vi "Init reg run.vi"() -> (1 "Rég acqui":T1(array[cluster]))   [LabVIEW 2022 SP3]
uses:
  Variables globales/Variables glob EUROTHERM.vi
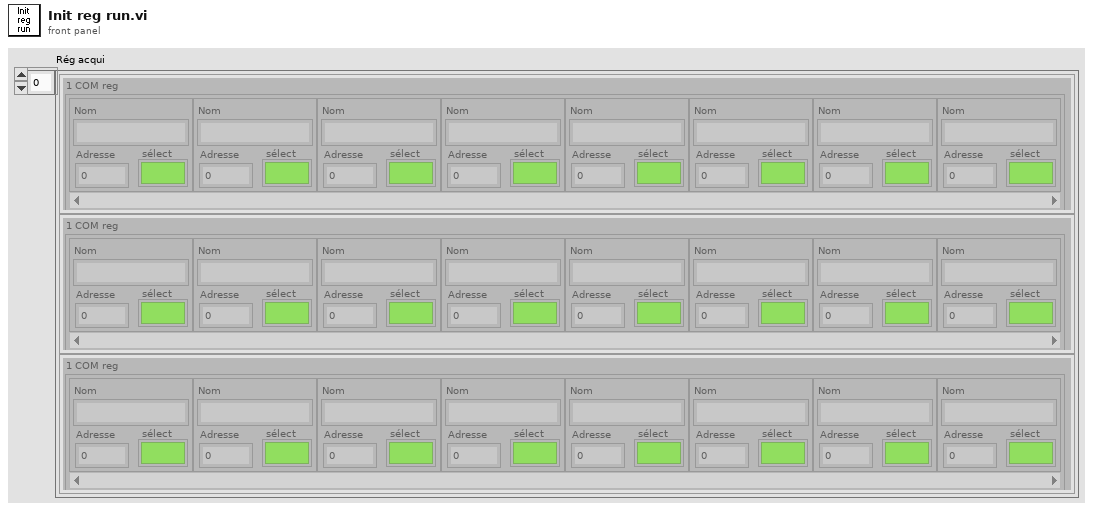
[diagram p1: front panel]
types:
  T1 = cluster{"1 COM reg":cluster{"Nom":string, "Adresse":u8, "sélect":bool}[]}[]
  T2 = cluster{"Noms voies select acqui 1COM":string[]}[]
  T3 = cluster{"1 COM reg":cluster{"Nom":string, "Adresse":u8, "sélect":bool}[]}
  T4 = cluster{"Nom":string, "Adresse":u8, "sélect":bool}[]
  T5 = cluster{"Nom":string, "Adresse":u8, "sélect":bool}
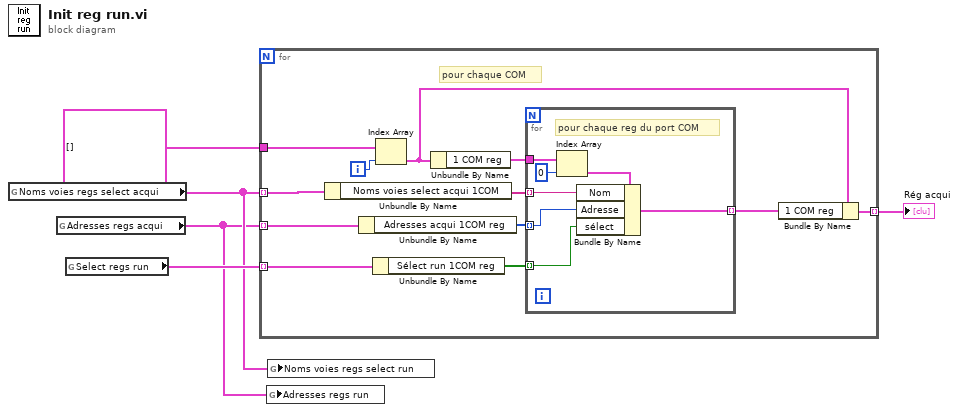
[diagram p0: block diagram]
diagram:
  n1 = global read "Variables glob EUROTHERM.vi" "Noms voies regs select acqui"() -> (w2:T2)
  n2 = global read "Variables glob EUROTHERM.vi" "Adresses regs acqui"() -> (w1:cluster{"Adresses acqui 1COM reg":u16[]}[])
  n3 = global read "Variables glob EUROTHERM.vi" "Select regs run"() -> (w3:cluster{"Sélect run 1COM reg":bool[]}[])
  n4 = for {
    tunnel: w2 -> [w11] mode=indexing
    tunnel: w1 -> [w13] mode=indexing
    tunnel: T1 [] ("Rég dispo") -> [w15]
    tunnel: [w16] -> w5 mode=indexing
    tunnel: w3 -> [w7] mode=indexing
    i -> [w14]
    # "pour chaque COM"
    n5 = Unbundle By Name(w11) -> ("Noms voies select acqui 1COM"=w10:string[])
    n6 = Unbundle By Name(w13) -> ("Adresses acqui 1COM reg"=w12:u16[])
    n7 = Unbundle By Name(w7) -> ("Sélect run 1COM reg"=w6:bool[])
    n8 = Index Array(array=w15, index=w14) -> (element=w8:T3)
    n9 = Unbundle By Name(w8) -> ("1 COM reg"=w17:T4)
    n10 = for {
      tunnel: w17 -> [w23]
      tunnel: w10 -> [w24] mode=indexing
      tunnel: w12 -> [w21] mode=indexing
      tunnel: [w20] -> w9 mode=indexing
      tunnel: w6 -> [w18] mode=indexing
      # "pour chaque reg du port COM"
      n11 = Index Array(array=w23, index=0 ("indice")) -> (element=w19:T5)
      n12 = Bundle By Name(cluster=w19, "Nom"=w24, "Adresse"=w21, "sélect"=w18) -> (w20:T5)
    }
    n13 = Bundle By Name(cluster=w8, "1 COM reg"=w9) -> (w16:T3)
  }
  "Rég acqui" <- w5
  n14 = global write "Variables glob EUROTHERM.vi" "Adresses regs run"(w1) -> ()
  n15 = global write "Variables glob EUROTHERM.vi" "Noms voies regs select run"(w2) -> ()
